vi "midiInClose.vi"(8 "error in":errorcluster, 11 "midi in":refnum<class "midi.lvclass">) -> (0 "error out":errorcluster, 3 "midi out":refnum<class "midi.lvclass">)   [LabVIEW 2020, in "midi.lvclass"]
doc: "The midiInClose function closes the specified MIDI input device."
uses:
  midi.lvclass
  midi.lvclass/midi.ctl
  cpp-src/MIDIInToLabVIEWWrapper/x64/Release/MIDIInToLabVIEWWrapper.dll
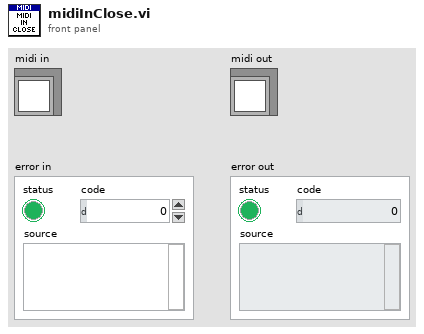
[diagram p1: front panel]
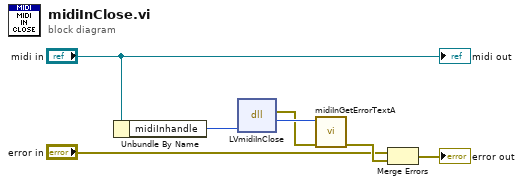
[diagram p0: block diagram]
diagram:
  n1 = Unbundle By Name("midi in") -> ("midiInhandle"=w4:u64)
  n2 = dll-call lib="C:/code/LabVIEW-MIDI/cpp-src/MIDIInToLabVIEWWrapper/x64/Release/MIDIInToLabVIEWWrapper.dll" fn="LVmidiInClose"("hMidiIn"=w4) -> (error out=w2:errorcluster, "error"=w3:i32)  [unwired: 4 in, 1 out]
  n3 = call "midiInGetErrorTextA.vi"("error in"=w2, "Error Code"=w3) -> ("error out"=w6:errorcluster)  [unwired: 9 in]
  n4 = Merge Errors("error in", w6) -> (→"error out":errorcluster)
  "midi out" <- "midi in"
